vi "CoolProp.vi"(6 "Fluid":string="Water", 7 "Output":string="T", 8 "Value2":dbl=1.0, 9 "Input Variable #2":enum16{"P [kPa]", "Q [-]", "D [kg/m^3]"}(ring)=enum."Q [-]", 10 "Value1":dbl=400.0, 11 "Input Variable #1":T1(ring)) -> (0 "error_message":string, 3 "Return Value":dbl=416.75835925510785)   [LabVIEW 2011]
uses:
  CoolProp.dll
  Desktop/CoolProp.dll
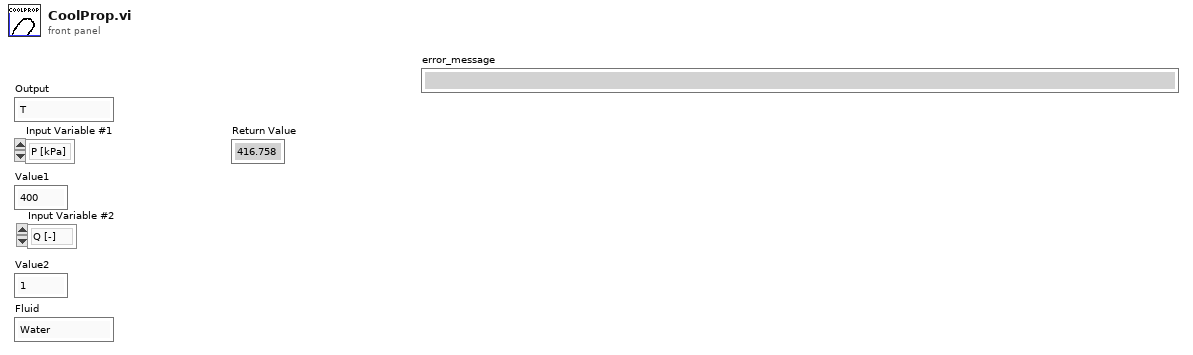
[diagram p1: front panel]
types:
  T1 = enum16{"P [kPa]", "T [K]", "S [kJ/kg/K]", "H [kJ/kg]"}
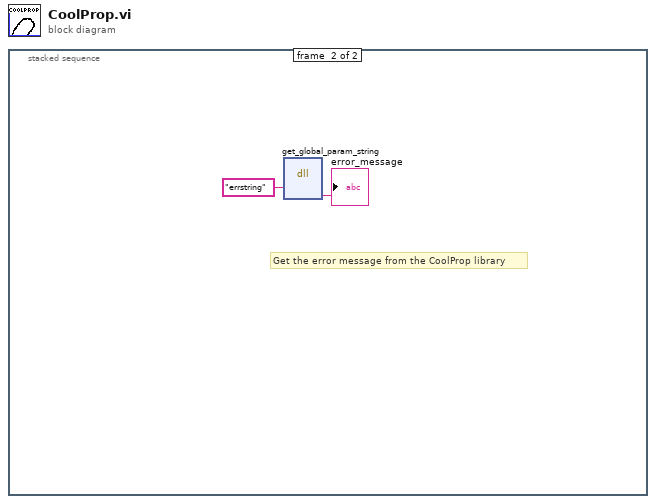
[diagram p0: block diagram]
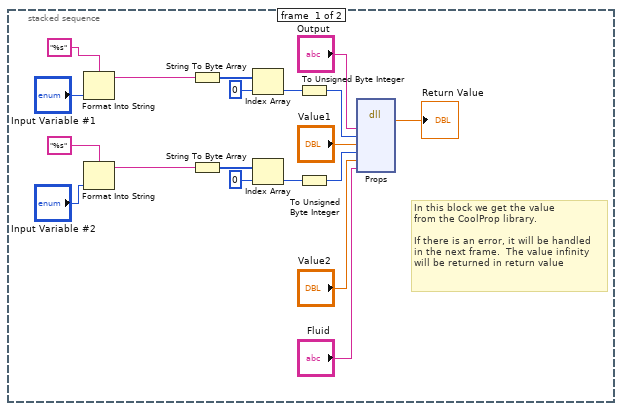
[diagram p2: hidden frame]
diagram:
  n1 = stacked-sequence {
    frame #0 {
      # "In this block we get the value\nfrom the CoolProp library.\n\nIf there is an error, it will be handled\nin the next frame.  The value infinity \nwill be returned in return value"
      n2 = Format Into String "Format Into String"(format string="%s", "Input Variable #1") -> (resulting string=w15:string)  [unwired: 2 in, 1 out]
      n3 = Format Into String "Format Into String"(format string="%s", "Input Variable #2") -> (resulting string=w19:string)  [unwired: 2 in, 1 out]
      n4 = String To Byte Array(string=w15) -> (unsigned byte array=w13:u8[])
      n5 = String To Byte Array(string=w19) -> (unsigned byte array=w7:u8[])
      n6 = Index Array(array=w13, index=0) -> (element=w12:u8)
      n7 = Index Array(array=w7, index=0) -> (element=w8:u8)
      n8 = To Unsigned Byte Integer(number=w12) -> (unsigned 8bit integer=w10:u8)
      n9 = To Unsigned Byte Integer(number=w8) -> (unsigned 8bit integer=w9:u8)
      n10 = dll-call lib="C:/Users/ian/Desktop/CoolProp.dll" fn="Props"("Output"="Output", "Input1"=w10, "Value1"="Value1", "Input2"=w9, "Value2"="Value2", "Fluid"="Fluid") -> ("OutputValue"=→"Return Value":dbl)  [unwired: 9 in, 2 out]
    }
    frame #1 {
      # "Get the error message from the CoolProp library"
      n11 = dll-call lib="C:/Users/ian/Desktop/CoolProp.dll" fn="get_global_param_string"("param"="errstring") -> ("error_message"=→"error_message":string)  [unwired: 4 in, 4 out]
    }
  }
